vi "Generate Simulated Data.vi"(8 "error in (no error)":errorcluster, 11 "Signal Type":T1) -> (0 "error out":errorcluster, 2 "Graph Data":waveform(dbl)[](array[waveform]))   [LabVIEW 2017, in "Acquisition.lvlib"]
doc: "Generates sample waveforms according to the signal type in the HW Config input."
uses:
  Acquisition.lvlib
  Signal Type.ctl
panel:
  # "Connector Pane"
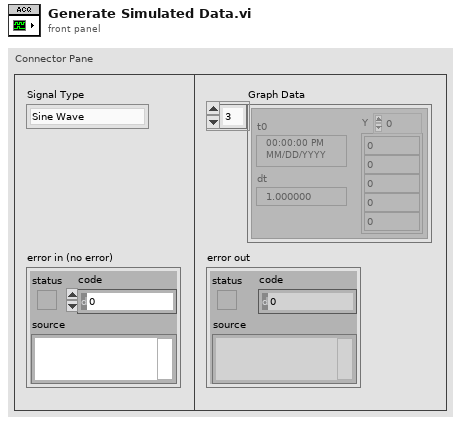
[diagram p1: front panel]
types:
  T1 = typedef "Acquisition.lvlib/Signal Type.ctl" = enum16{"Sine Wave", "Square with Noise"}
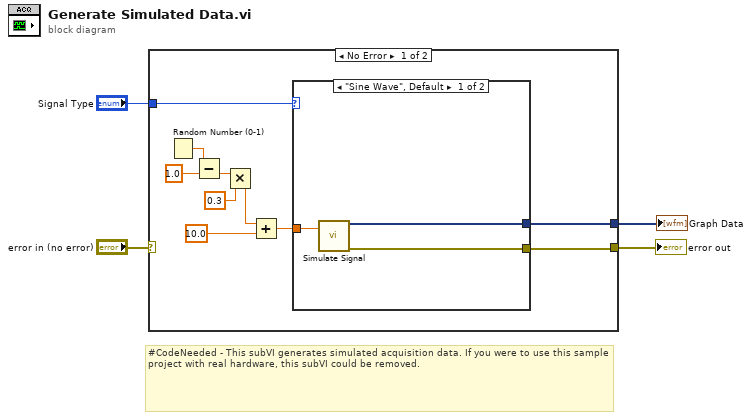
[diagram p0: block diagram]
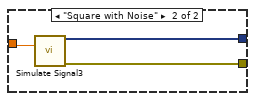
[diagram p2: hidden frame]
diagram:
  # "#CodeNeeded - This subVI generates simulated acquisition data. If you were to use this sample project with real hardware, this subVI could be removed."
  n1 = case shown="No Error" "error in (no error)" {
    selector: "error in (no error)" -> [_ w21]
    tunnel: [w6 w21] -> w3
    tunnel: "Signal Type" -> [w14 _]
    tunnel: [w5 _] -> w1
    frame No Error {
      n2 = Random Number (0-1)() -> (number: 0 to 1=w12:dbl)
      n3 = Subtract(x=w12, y=1.0) -> (x-y=w11:dbl)
      n4 = Multiply(x=w11, y=0.3) -> (x*y=w13:dbl)
      n5 = Add(x=w13, y=10.0 ("Frequency")) -> (x+y=w7:dbl)
      n6 = case shown="\"Sine Wave\", Default" w14 {
        tunnel: w7 -> [w17 w20]
        tunnel: [w16 w19] -> w5
        tunnel: [w15 w18] -> w6
        frame "Sine Wave", Default {
          n7 = call "Simulate Signal"("Frequency"=w17) -> ("Sine with Gaussian Noise"=w16:dynamicdata, "error out"=w15:errorcluster)  [unwired: 13 in]
        }
        frame "Square with Noise" {
          n8 = call "Simulate Signal3"("Frequency"=w20) -> ("Square with Gaussian Noise"=w19:dynamicdata, "error out"=w18:errorcluster)  [unwired: 13 in]
        }
      }
    }
    frame Error {
    }
  }
  "error out" <- w3
  "Graph Data" <- w1
